vi "Delete Item from LVClass.vi"(7 "Item Type":string="VI", 8 "error in (no error)":errorcluster, 10 "Item name":string, 11 "LVClassLibrary in":refnum<vi>) -> (0 "error out":errorcluster, 2 "Deleted ?":bool, 3 "LVClassLibrary out":refnum<vi>)   [LabVIEW 2019, in "gRPC Template Creation Utility.lvlib"]
uses:
  gRPC Template Creation Utility.lvlib
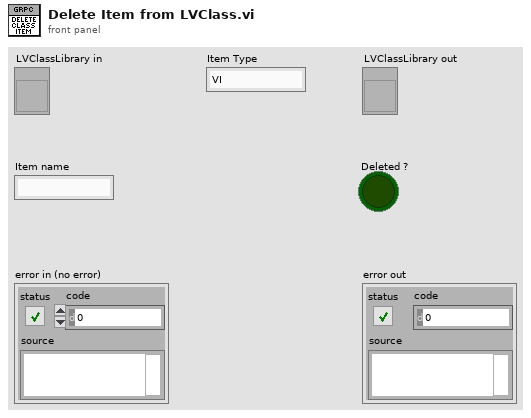
[diagram p1: front panel]
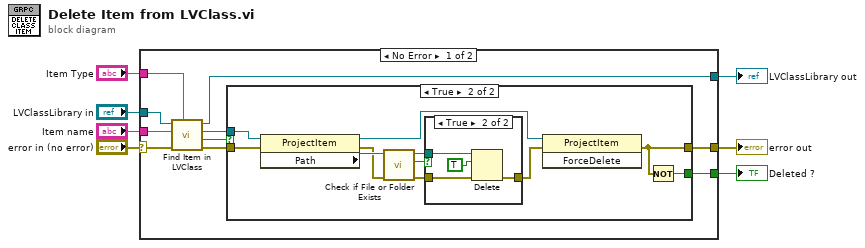
[diagram p0: block diagram]
diagram:
  n1 = case shown="No Error" "error in (no error)" {
    selector: "error in (no error)" -> [w10 w36]
    tunnel: [w17 w35] -> w7
    tunnel: "Item name" -> [w16 _]
    tunnel: "LVClassLibrary in" -> [w15 w35]
    tunnel: "Item Type" -> [w14 _]
    tunnel: [w9 w36] -> w2
    tunnel: [w8 _] -> w1
    frame No Error {
      n2 = call "Find Item in LVClass.vi"("Item Type"=w14, "error in (no error)"=w10, "Item Name"=w16, "Class Item in"=w15) -> ("error out"=w11:errorcluster, "Found?"=w13:bool, "Project Item (Class Item)"=w12:refnum<vi>, "Class Item out"=w17:refnum<vi>)  [unwired: 4 in]
      n3 = case shown="True" w13 {
        tunnel: w12 -> [_ w29]
        tunnel: w11 -> [w18 w24]
        tunnel: [w18 w28] -> w9
        tunnel: [_ w27] -> w8
        frame False {
        }
        frame True {
          n4 = property class="ProjectItem"(reference=w29, error in=w24) -> (reference out=w25:refnum<vi>, error out=w22:errorcluster, "Path"=w23:path)
          n5 = call <vilib>:"Check if File or Folder Exists.vi"("error in (no error)"=w22, "path"=w23) -> ("error out"=w20:errorcluster, "file or folder exists?"=w26:bool, "dup path"=w21:path)  [unwired: 7 in]
          n6 = case shown="True" w26 {
            tunnel: w21 -> [_ w34]
            tunnel: w20 -> [w30 w33]
            tunnel: [w30 w32] -> w19
            frame False {
            }
            frame True {
              n7 = Delete(path (use dialog)=w34, entire hierarchy (F)=TRUE, error in=w33) -> (error out=w32:errorcluster)  [unwired: 2 in, 2 out]
            }
          }
          n8 = invoke class="ProjectItem" method="ForceDelete"(reference=w25, error in=w19) -> (error out=w28:errorcluster)  [unwired: 1 in, 2 out]
          n9 = Not(x=w28) -> (.not. x?=w27:bool)
        }
      }
    }
    frame Error {
    }
  }
  "LVClassLibrary out" <- w7
  "error out" <- w2
  "Deleted ?" <- w1
